vi "Reading_Visa.vi"(10 "Numeric":i32) -> (3 "output array":string[][](array[string]))   [LabVIEW 2024]
uses:
  <vilib>/Instr/_visa.llb/VISA Configure Serial Port (Instr).vi
panel:
  in  "VISA resource name":refnum<visa-resource-name>="COM6"
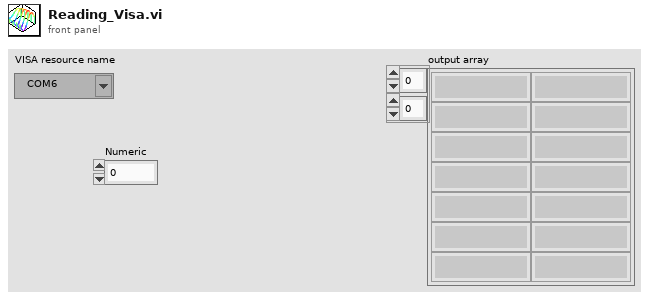
[diagram p1: front panel]
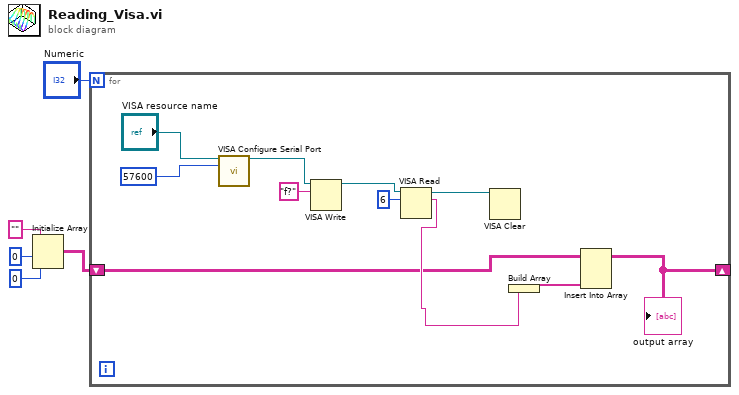
[diagram p0: block diagram]
diagram:
  n1 = Initialize Array "Initialize Array"("", 0 ("dimension size"), 0 ("dimension size")) -> (w2:string[][])
  n2 = for {
    N: "Numeric" -> [_]
    shift-right: [w6] -> _
    shift-left: w2 -> [w7]
    n3 = call-poly "VISA Configure Serial Port"("VISA resource name"="VISA resource name", "baud rate (9600)"=u32 57600) -> ("VISA resource name out"=w12:refnum<visa-resource-name>)  [unwired: 12 in, 1 out]
    n4 = VISA Write(VISA resource name=w12, write buffer="f?") -> (VISA resource name out=w13:refnum<visa-resource-name>)  [unwired: 1 in, 2 out]
    n5 = VISA Read(VISA resource name=w13, byte count=u32 6) -> (VISA resource name out=w14:refnum<visa-resource-name>, read buffer=w8:string)  [unwired: 1 in, 2 out]
    n6 = VISA Clear(VISA resource name=w14) -> ()  [unwired: 1 in, 2 out]
    n7 = Build Array(w8) -> (w9:string[])
    n8 = Insert Into Array(array=w7, new element=w9) -> (w6:string[][])  [unwired: 2 in]
    "output array" <- w6
  }
